vi "SolutionBuilder.vi"(6 "CLI Arguments":string[](array[string]), 7 "Preview?":bool, 8 "Version":T1, 9 "Log file path":path, 10 "Rebuild?":bool, 11 "Path":path) -> (0 "error out":errorcluster, 1 "Generated file":T3, 2 "Successful builds":T2[](array[typedef]), 3 "status":bool)   [LabVIEW 2019]
uses:
  SolutionBuilder/BuildManager/GeneratedFile.ctl
  SolutionBuilder/BuildManager/BuildProjectInfo.ctl
  SolutionBuilder/SolutionBuilder.lvclass
  SolutionBuilder/SolutionBuilder.lvclass/SolutionBuilder.ctl
  SolutionBuilder/SolutionBuilder.lvlib
  SolutionBuilder/BuildManager/BuildManager.lvclass
panel:
  in  "Cancel build":bool
  out "source":string
  out "code":i32
  out "Results":i32(listbox)=-1
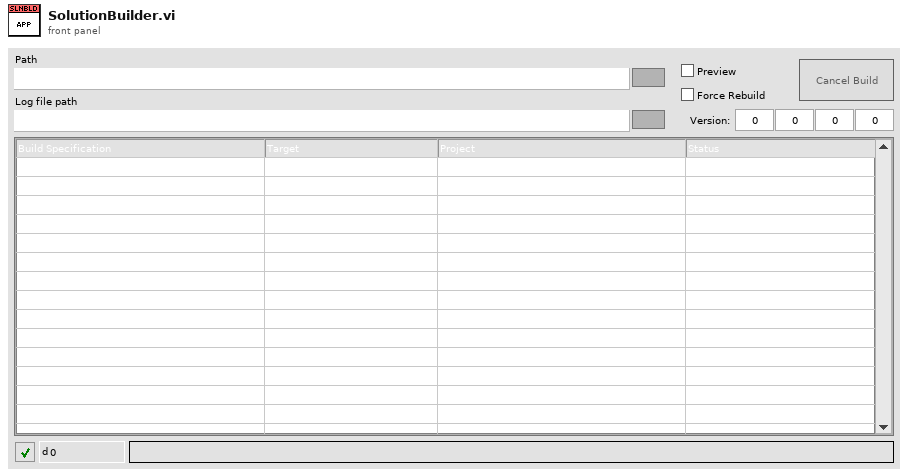
[diagram p1: front panel]
types:
  T1 = cluster{"Version:":u16, "minor":u16, "fix":u16, "build":u16}
  T2 = typedef "SolutionBuilder.lvlib/BuildManager.lvclass/BuildProjectInfo.ctl" = cluster{"Project path":string, "Build spec name":string, "Target":string, "Version string":string}
  T3 = typedef "SolutionBuilder.lvlib/BuildManager.lvclass/GeneratedFile.ctl" = map{T2, set{string}}
  T4 = typedef "SolutionBuilder.lvlib/Events.ctl" = cluster{"UpdateList":T5, "ItemBuilt":T6, "Stop":refnum<user-event>}
  T5 = typedef "SolutionBuilder.lvlib/EventUpdateList.ctl" = refnum<user-event>
  T6 = typedef "SolutionBuilder.lvlib/EventItemBuilt.ctl" = refnum<user-event>
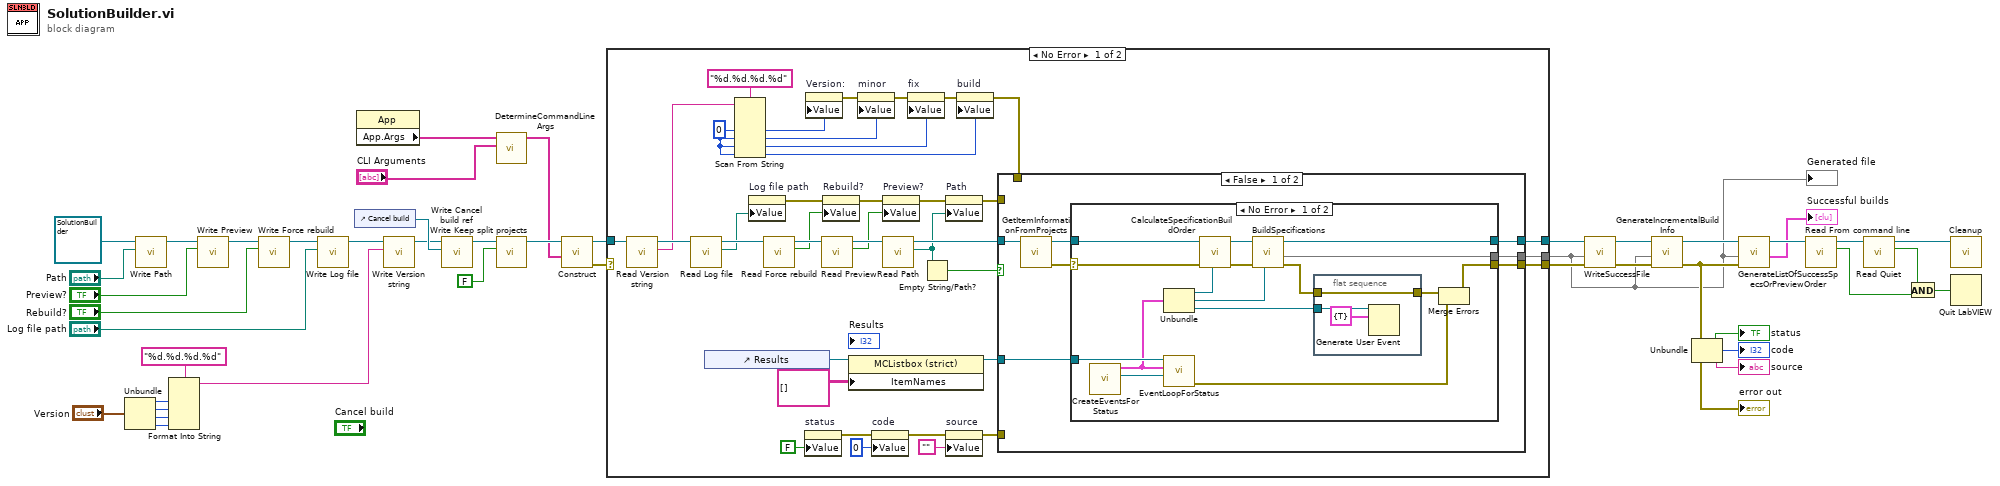
[diagram p0: block diagram]
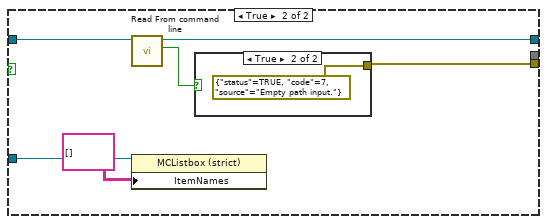
[diagram p3: hidden frame]
diagram:
  n1 = Unbundle("Version") -> ("Version:"=w5:u16, "minor"=w4:u16, "fix"=w3:u16, "build"=w2:u16)
  n2 = call "Write Path.vi"("Path"="Path", "SolutionBuilder in"=refnum<class "SolutionBuilder.lvclass"> refnum) -> ("SolutionBuilder out"=w43:refnum<class "SolutionBuilder.lvclass">)  [unwired: 9 in]
  n3 = Format Into String(format string="%d.%d.%d.%d", w5, w4, w3, w2) -> (resulting string=w8:string)  [unwired: 2 in, 1 out]
  n4 = call "Write Preview.vi"("Preview?"="Preview?", "SolutionBuilder in"=w43) -> ("SolutionBuilder out"=w28:refnum<class "SolutionBuilder.lvclass">)  [unwired: 9 in]
  n5 = call "Write Force rebuild.vi"("Force rebuild"="Rebuild?", "SolutionBuilder in"=w28) -> ("SolutionBuilder out"=w24:refnum<class "SolutionBuilder.lvclass">)  [unwired: 9 in]
  n6 = call "Write Log file.vi"("Log file"="Log file path", "SolutionBuilder in"=w24) -> ("SolutionBuilder out"=w10:refnum<class "SolutionBuilder.lvclass">)  [unwired: 9 in]
  n7 = control-ref of="Cancel build"() -> (w29:refnum<vi>)
  n8 = property class="App"() -> ("App.Args"=w18:string[])  [unwired: 2 in, 2 out]
  n9 = call "Write Version string.vi"("Version string"=w8, "SolutionBuilder in"=w10) -> ("SolutionBuilder out"=w9:refnum<class "SolutionBuilder.lvclass">)  [unwired: 9 in]
  n10 = call "Write Cancel build ref.vi"("Cancel build ref"=w29, "SolutionBuilder in"=w9) -> ("SolutionBuilder out"=w22:refnum<class "SolutionBuilder.lvclass">)  [unwired: 9 in]
  n11 = call "DetermineCommandLineArgs.vi"("CLI Arguments"="CLI Arguments", "App.Args in"=w18) -> ("App.Args out"=w17:string[])  [unwired: 9 in]
  n12 = call-dynamic "Write Keep split projects.vi"("Keep split projects?"=FALSE, "SolutionBuilder in"=w22) -> ("SolutionBuilder out"=w21:refnum<class "SolutionBuilder.lvclass">)  [unwired: 9 in]
  n13 = call "Construct.vi"("App.Args"=w17, "SolutionBuilder in"=w21) -> ("error out"=w1:errorcluster, "SolutionBuilder out"=w7:refnum<class "SolutionBuilder.lvclass">)  [unwired: 8 in]
  n14 = case shown="No Error" w1 {
    selector: w1 -> [_ w117]
    tunnel: [w71 w118] -> w31
    tunnel: [w70 w117] -> w30
    tunnel: [w57 _] -> w12
    tunnel: w7 -> [w56 w118]
    frame No Error {
      w50 = u16 0 ("default value 1")
      n15 = call "Read Version string.vi"("SolutionBuilder in"=w56) -> ("Version string"=w49:string, "SolutionBuilder out"=w55:refnum<class "SolutionBuilder.lvclass">)  [unwired: 9 in]
      n16 = call "Read Log file.vi"("SolutionBuilder in"=w55) -> ("Log file"=w58:path, "SolutionBuilder out"=w60:refnum<class "SolutionBuilder.lvclass">)  [unwired: 9 in]
      n17 = control-ref of="Results"() -> (w74:refnum<vi>)
      n18 = Scan From String(format string="%d.%d.%d.%d", input string=w49, default 1=w50, default 2=w50, default 3=w50, default 4=w50) -> (output 1=w48:u16, output 2=w47:u16, output 3=w46:u16, output 4=w45:u16)  [unwired: 2 in, 3 out]
      n19 = property on="Log file path" class="Path"("Value"=w58) -> (error out=w59:errorcluster)  [unwired: 2 in, 1 out]
      n20 = call "Read Force rebuild.vi"("SolutionBuilder in"=w60) -> ("Force rebuild"=w62:bool, "SolutionBuilder out"=w63:refnum<class "SolutionBuilder.lvclass">)  [unwired: 9 in]
      n21 = property on="status" class="Bool (strict)"("Value"=FALSE ("status")) -> (error out=w69:errorcluster)  [unwired: 2 in, 1 out]
      n22 = property on="Version:" class="DigNum (strict)"("Value"=w48) -> (error out=w54:errorcluster)  [unwired: 2 in, 1 out]
      n23 = call "Read Preview.vi"("SolutionBuilder in"=w63) -> ("Preview?"=w75:bool, "SolutionBuilder out"=w79:refnum<class "SolutionBuilder.lvclass">)  [unwired: 9 in]
      n24 = property on="Rebuild?" class="Bool (strict)"(error in=w59, "Value"=w62) -> (error out=w61:errorcluster)  [unwired: 1 in, 1 out]
      n25 = property class="MCListbox (strict)"(reference=w74, "ItemNames"=string[][] [] ("Item Names")) -> (reference out=w73:refnum<vi>)  [unwired: 1 in, 1 out]
      n26 = property on="minor" class="DigNum (strict)"(error in=w54, "Value"=w47) -> (error out=w53:errorcluster)  [unwired: 1 in, 1 out]
      n27 = property on="code" class="DigNum (strict)"(error in=w69, "Value"=0 ("code")) -> (error out=w68:errorcluster)  [unwired: 1 in, 1 out]
      n28 = property on="Preview?" class="Bool (strict)"(error in=w61, "Value"=w75) -> (error out=w76:errorcluster)  [unwired: 1 in, 1 out]
      n29 = call "Read Path.vi"("SolutionBuilder in"=w79) -> ("Path"=w78:path, "SolutionBuilder out"=w80:refnum<class "SolutionBuilder.lvclass">)  [unwired: 9 in]
      n30 = property on="fix" class="DigNum (strict)"(error in=w53, "Value"=w46) -> (error out=w52:errorcluster)  [unwired: 1 in, 1 out]
      n31 = Empty String/Path?(string/path=w78) -> (empty?=w81:bool)
      n32 = property on="Path" class="Path"(error in=w76, "Value"=w78) -> (error out=w77:errorcluster)  [unwired: 1 in, 1 out]
      n33 = property on="source" class="Str"(error in=w68, "Value"="") -> (error out=w64:errorcluster)  [unwired: 1 in, 1 out]
      n34 = property on="build" class="DigNum (strict)"(error in=w52, "Value"=w45) -> (error out=w51:errorcluster)  [unwired: 1 in, 1 out]
      n35 = case shown="False" w81 {
        tunnel: [w88 w115] -> w70
        tunnel: w73 -> [w87 w113]
        tunnel: w80 -> [w83 w111]
        tunnel: [w86 w112] -> w71
        tunnel: w77 -> [_ _]
        tunnel: [w82 _] -> w57
        tunnel: w64 -> [_ _]
        tunnel: w51 -> [_ _]
        frame False {
          n36 = call "GetItemInformationFromProjects.vi"("SolutionBuilder in"=w83) -> ("error out"=w84:errorcluster, "SolutionBuilder out"=w85:refnum<class "SolutionBuilder.lvclass">)  [unwired: 9 in]
          n37 = case shown="No Error" w84 {
            selector: w84 -> [w94 w108]
            tunnel: w87 -> [w98 _]
            tunnel: w85 -> [w97 w109]
            tunnel: [w96 w109] -> w86
            tunnel: [w95 w108] -> w88
            tunnel: [w89 _] -> w82
            frame No Error {
              n38 = call "CreateEventsForStatus.vi"() -> ("Event Registration Refnum"=w90:refnum<event-registration>, "Events"=w91:T4)  [unwired: 10 in]
              n39 = Unbundle(w91) -> ("UpdateList"=w104:T5, "ItemBuilt"=w101:T6, "Stop"=w102:refnum<user-event>)
              n40 = call "EventLoopForStatus.vi"("Event Registration Refnum"=w90, "Events"=w91, "MulticolumnListbox in"=w98) -> ("error out"=w103:errorcluster)  [unwired: 8 in]
              n41 = call "CalculateSpecificationBuildOrder.vi"("UpdateList"=w104, "error in (no error)"=w94, "SolutionBuilder in"=w97) -> ("error out"=w100:errorcluster, "SolutionBuilder out"=w99:refnum<class "SolutionBuilder.lvclass">)  [unwired: 7 in]
              n42 = call "BuildSpecifications.vi"("ItemBuilt"=w101, "error in (no error)"=w100, "SolutionBuilder in"=w99) -> ("error out"=w92:errorcluster, "Generated file"=w89:T3, "SolutionBuilder out"=w96:refnum<class "SolutionBuilder.lvclass">)  [unwired: 6 in]
              n43 = flat-sequence {
                tunnel: w102 -> [w106]
                tunnel: [w105] -> w93
                tunnel: w92 -> [w105]
                frame #0 {
                  n44 = Generate User Event(user event=w106, event data cluster=cluster{"Stop":bool} {"Stop"=TRUE} ("event data")) -> ()  [unwired: 2 in, 2 out]
                }
              }
              n45 = Merge Errors(w93, w103) -> (w95:errorcluster)
            }
            frame Error {
            }
          }
        }
        frame True {
          n46 = call "Read From command line.vi"("SolutionBuilder in"=w111) -> ("From command line?"=w110:bool, "SolutionBuilder out"=w112:refnum<class "SolutionBuilder.lvclass">)  [unwired: 9 in]
          n47 = property class="MCListbox (strict)"(reference=w113, "ItemNames"=string[][] [] ("Item Names")) -> ()  [unwired: 1 in, 2 out]
          n48 = case shown="True" w110 {
            tunnel: [_ errorcluster {"status"=TRUE, "code"=7, "source"="Empty path input."} ("t")] -> w115
            frame False {
            }
            frame True {
            }
          }
        }
      }
    }
    frame Error {
    }
  }
  "Generated file" <- w12
  n49 = call "WriteSuccessFile.vi"("error in (no error)"=w30, "Generated file"=w12, "SolutionBuilder in"=w31) -> ("error out"=w25:errorcluster, "SolutionBuilder out"=w26:refnum<class "SolutionBuilder.lvclass">)  [unwired: 7 in]
  n50 = call "GenerateIncrementalBuildInfo.vi"("error in (no error)"=w25, "Generated file"=w12, "SolutionBuilder in"=w26) -> ("error out"=w14:errorcluster, "SolutionBuilder out"=w16:refnum<class "SolutionBuilder.lvclass">)  [unwired: 7 in]
  "error out" <- w14
  n51 = Unbundle(w14) -> ("status"=→"status":bool, "code"=→"code":i32, "source"=→"source":string)
  n52 = call "GenerateListOfSuccessSpecsOrPreviewOrder.vi"("error in (no error)"=w14, "Generated file"=w12, "SolutionBuilder in"=w16) -> ("Builds"=→"Successful builds":T2[], "SolutionBuilder out"=w15:refnum<class "SolutionBuilder.lvclass">)  [unwired: 6 in, 1 out]
  n53 = call "Read From command line.vi"("SolutionBuilder in"=w15) -> ("From command line?"=w33:bool, "SolutionBuilder out"=w35:refnum<class "SolutionBuilder.lvclass">)  [unwired: 9 in]
  n54 = call "Read Quiet.vi"("SolutionBuilder in"=w35) -> ("Quiet?"=w34:bool, "SolutionBuilder out"=w39:refnum<class "SolutionBuilder.lvclass">)  [unwired: 9 in]
  n55 = And(x=w34, y=w33) -> (x .and. y?=w32:bool)
  n56 = call "Cleanup.vi"("SolutionBuilder in"=w39) -> ()  [unwired: 9 in, 2 out]
  n57 = Quit LabVIEW(quit? (T)=w32) -> ()
